vi "Measurement Logic.vi"(8 "error in":errorcluster, 9 "measurement configuration":T4={"config"="SI1", "BITFILE"=""}, 10 "measure call context in":refnum<class "Measure Call Context.lvclass">, 11 "user event out":refnum<user-event>) -> (0 "Error Out":errorcluster, 2 "measure call context out":refnum<class "Measure Call Context.lvclass">, 3 "measurement results":T1 {"BYTES ACQUIRED" format="%#.6p"})   [LabVIEW 2025, in "Automotive Vision.lvclass"]
doc: "Contains the core logic for executing the measurement."
uses:
  Automotive Vision.lvclass
  <vilib>/Plug-In SDKs/Measurements/Measure Call Context/Measure Call Context.lvclass
  <vilib>/rvi/interface/nirviCloseFPGA/nirviCloseFPGA.xnode
  Automotive Vision.lvclass/Automotive Vision.ctl
  Measurement Results.ctl
  ttashjia/GSE/Host/Acq/GettingStarted_Acq_148X_Host.lvlib
  ttashjia/GSE/Host/Common/GettingStarted_Common_148X_Host.lvlib
  <instrlib>/FlexRIO/API/Host/v1/NI FlexRIO API v1.lvlib
  <vilib>/vision/Image Controls.llb/IMAQ Image.ctl
  <instrlib>/FlexRIO/CSI-2/v2/Common/Types/LLP Data Type.ctl
  <instrlib>/FlexRIO/CSI-2/v2/Common/NI CSI-2 API Common v2.lvlib
  <vilib>/FPGAPlugInAG/Dynamic/niLvFpga_Close_Dynamic.vi
  <instrlib>/FlexRIO/API/Host/v1/NI FlexRIO/API/Wait for PoC Safe to Disconnect Channels Array.vi
  Automotive-Vision OOB Data Transfer/Automotive-Vision OOB Data Transfer.lvlib
  Measurement Configuration.ctl
panel:
  in  "Serial Channel (2nd Display)":fxp<+,3,3>
  in  "Serial Channel (1st Display)":fxp<+,3,3>
  in  "Acquired Serial Input Channel Data":T2(tab)
  out "Source Rate (fps)(1st Display)":dbl
  out "Update Rate (fps)(1st Display)":dbl
  out "1st channel display":T3(plugin-control)
  out "Bytes Acquired (1st Channel)":i64 format="%#.6p"
  out "Packets Logged (1st Channel)":i64
  out "Source Rate (fps)(2nd Display)":dbl
  out "Update Rate (fps)(2nd Display)":dbl
  out "2nd channel display":T3(plugin-control)
  out "Packets Logged (2nd Channel)":i64
  out "Bytes Acquired (2nd Channel)":i64 format="%#.6p"
  out "Acquisition In Progress":bool
  out "Acquisition Duration (s)":dbl format="%.1f"
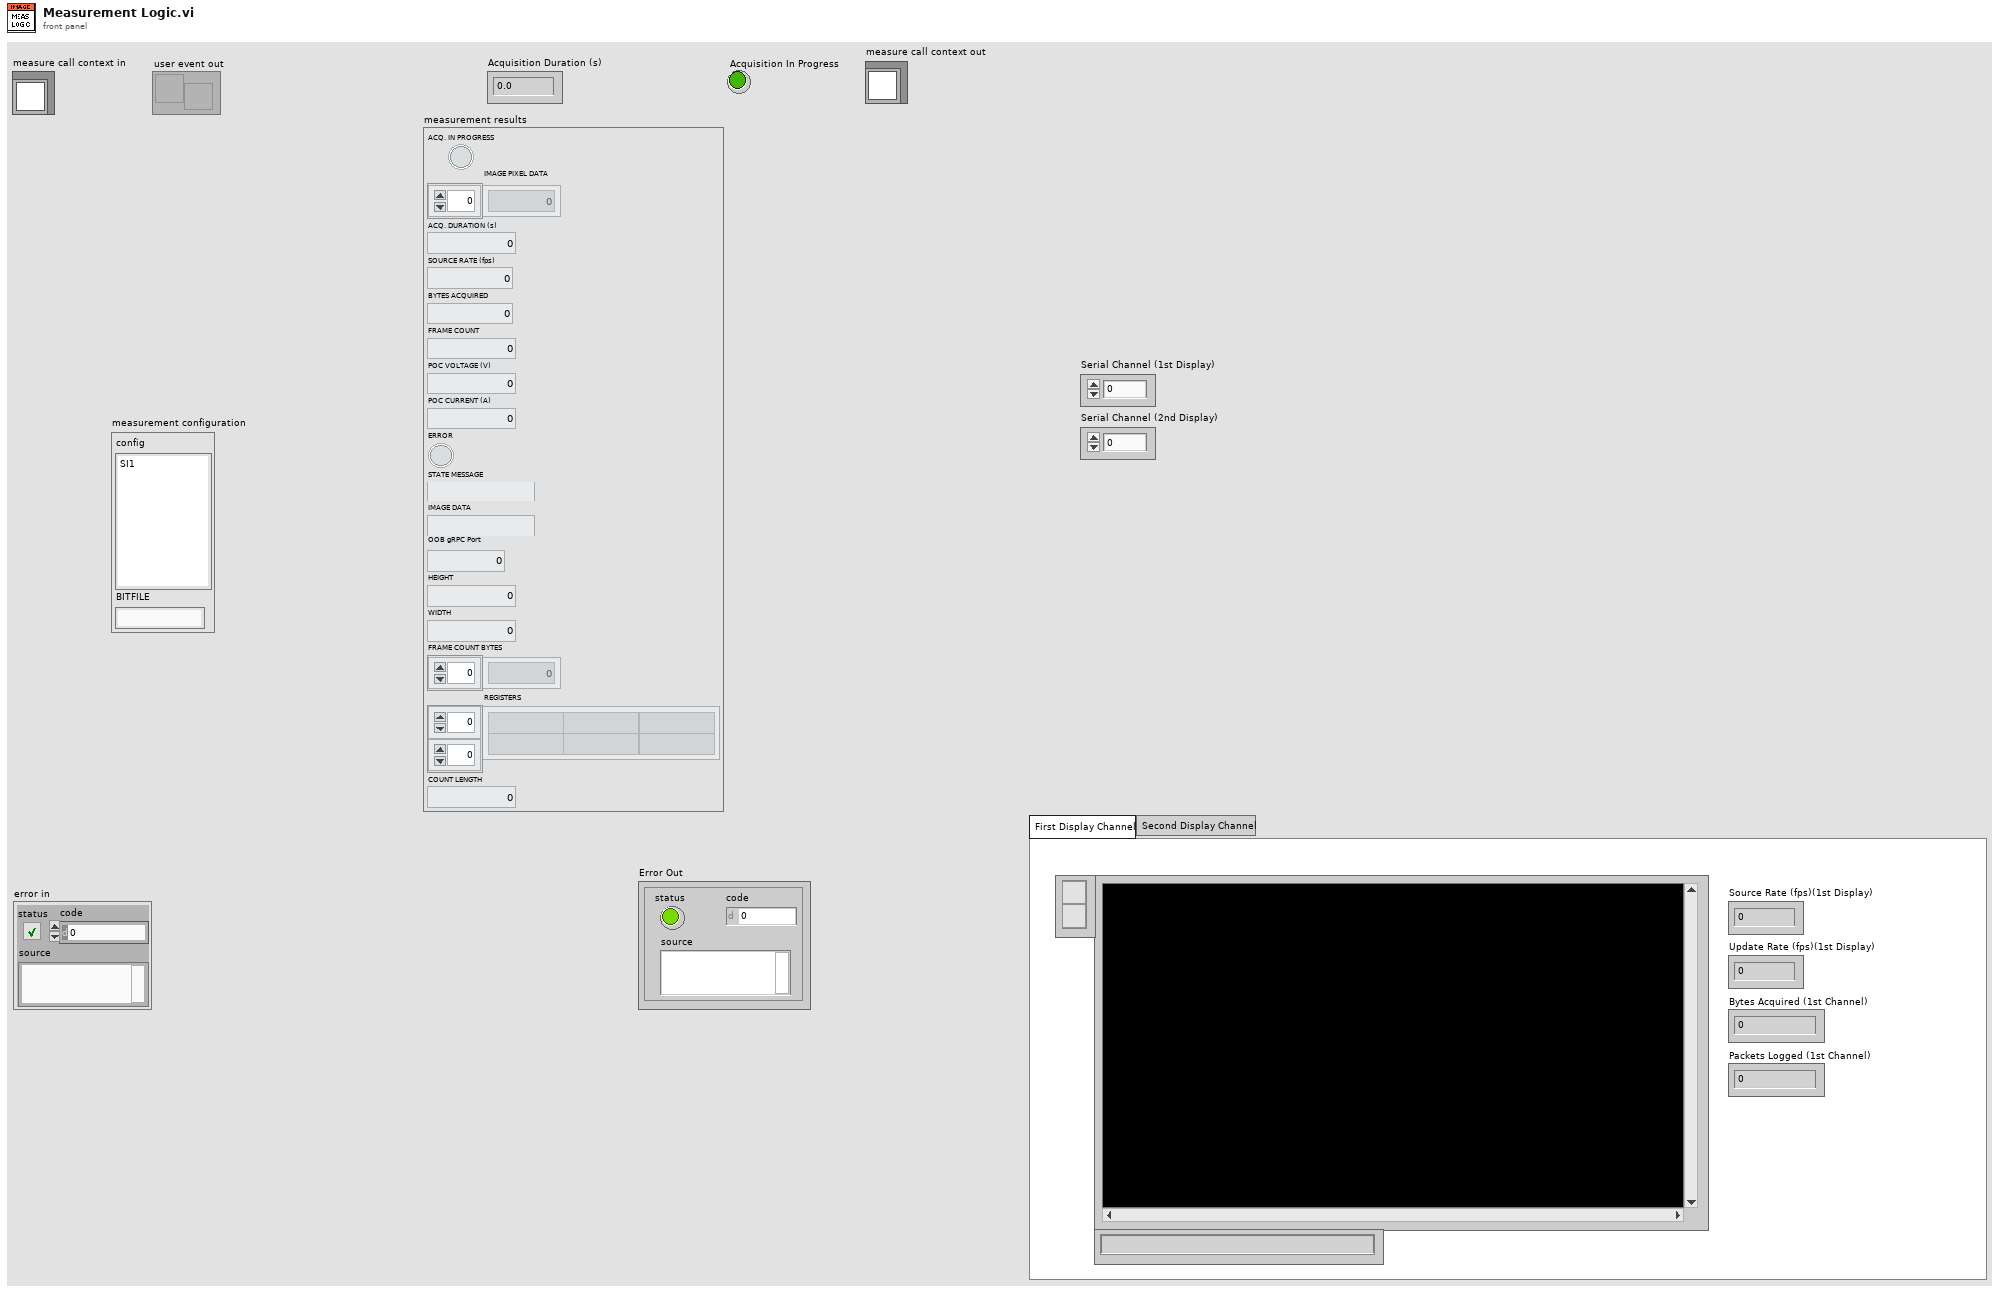
[diagram p1: front panel]
types:
  T1 = typedef "Automotive Vision.lvclass/Measurement Results.ctl" = cluster{"ACQ. IN PROGRESS":bool, "IMAGE PIXEL DATA":u32[], "ACQ. DURATION (s)":dbl, "SOURCE RATE (fps)":dbl, "BYTES ACQUIRED":u64, "FRAME COUNT":u64, "POC VOLTAGE (V)":dbl, "POC CURRENT (A)":dbl, "ERROR":bool, "STATE MESSAGE":string, "IMAGE DATA":string, "OOB gRPC Port":i32, "HEIGHT":u64, "WIDTH":u64, "FRAME COUNT BYTES":u32[], "REGISTERS":string[][], "COUNT LENGTH":u64}
  T2 = enum32{"First Display Channel", "Second Display Channel"}
  T3 = typedef "IMAQ Image.ctl" = refnum<image>
  T4 = typedef "Automotive Vision.lvclass/Measurement Configuration.ctl" = cluster{"config":string, "BITFILE":string}
  T5 = typedef "NI CSI-2 API Common v2.lvlib/LLP Data Type.ctl" = enum8{"Frame Start", "Frame End", "Line Start", "Line End", "End of Transmission", "Reserved 0", "Reserved 1", "Reserved 2", "Generic Short Packet 1", "Generic Short Packet 2", "Generic Short Packet 3", "Generic Short Packet 4", "Generic Short Packet 5", "Generic Short Packet 6", "Generic Short Packet 7", "Generic Short Packet 8", "Null", "Blanking Data", "Embedded 8-bit non Image Data", "Generic Long Packet 1", "Generic Long Packet 2", "Generic Long Packet 3", "Generic Long Packet 4", "Reserved 3", "YUV420 8-bit", "YUV420 10-bit", "Legacy YUV420 8-bit", "Reserved 4", "YUV420 8-bit Chroma Shifted", "YUV420 10-bit Chroma Shifted", "YUV422 8-bit", "YUV422 10-bit", "RGB444", "RGB555", "RGB565", "RGB666", "RGB888", "Reserved 5", "Reserved 6", "RAW 24", "RAW 6", "RAW 7", "RAW 8", "RAW 10", "RAW 12", "RAW 14", "RAW 16", "RAW 20", "User Defined 8-bit Data 1", "User Defined 8-bit Data 2", "User Defined 8-bit Data 3", "User Defined 8-bit Data 4", "User Defined 8-bit Data 5", "User Defined 8-bit Data 6", "User Defined 8-bit Data 7", "User Defined 8-bit Data 8", "USL Command", "Reserved 7", "Reserved 8", "Reserved 9", "Reserved 10", "Reserved 11", "Reserved 12", "LRTE EPD Spacer"}
  T6 = typedef "GettingStarted_Common_148X_Host.lvlib/Serial Channel Configuration.ctl" = cluster{"Serial Channel":string, "FPGA Display Parameters":T7, "RAW Display Parameters":cluster{"Interpretation":T8, "Bayer Parameters":cluster{"Pattern":i32, "Algorithm":i32, "Red Gain":dbl, "Green Gain":dbl, "Blue Gain":dbl}}}
  T7 = typedef "NI CSI-2 API FPGA v2.lvlib/Display Parameters.ctl" = cluster{"virtual channel":fxp<+,4,4>, "payload data type":T5, "frame skip count":u16, "line skip count":u8, "pixel skip count":fxp<+,5,5>}
  T8 = typedef "GettingStarted_Common_148X_Host.lvlib/RAW Interpretation for Display.ctl" = enum16{"Grayscale", "Bayer", "RGB", "YUV422", "YUV420", "Legacy YUV420"}
  T9 = typedef "Automotive Vision.lvclass/autovision_config.ctl" = cluster{"RIO Device":string, "Serial Channel":string, "SERDES Script":string, "POC Source":u32, "CSI-2 Data Source":u32, "Lane Count":u32, "Reference Clock":dbl, "Image Data Type":u32, "Interpretation":u32, "Pattern":u32, "Algorithm":u32, "Virtual Channel":u32, "Embedded Data":T10, "Registers":T12[], "Log Path":string}
  T10 = typedef "Automotive Vision.lvclass/embedded data.ctl" = cluster{"Pre-embedded Lines":dbl, "Pre-embedded Line Length":dbl, "Post-embedded Lines":dbl, "Post-embedded Line Length":dbl, "Frame Count":T11}
  T11 = typedef "Automotive Vision.lvclass/embedded data item.ctl" = cluster{"Line":dbl, "Offset":dbl, "Byte Count":dbl}
  T12 = typedef "Automotive Vision.lvclass/register.ctl" = cluster{"Name":string, "Device":u8, "Address":u16, "Min":u16, "Max":u16}
  T13 = typedef "GettingStarted_Common_148X_Host.lvlib/Serial Channel Display Parameters.ctl" = cluster{"images":cluster{"grayscale":T3, "color":T3}, "RAW parameters":cluster{"interpretation":T8, "bayer parameters":cluster{"pattern":i32, "algorithm":i32, "red gain":dbl, "green gain":dbl, "blue gain":dbl}}}
  T14 = typedef "Automotive-Vision OOB Data Transfer.lvlib/OOB to Logic Data.ctl" = cluster{"PauseResume":bool, "ExportPath":string, "ExportType":u16, "Export":bool}
  T15 = cluster{"Acquisition In Progress":refnum<vi>, "Acquisition Duration (s)":refnum<vi>, "Bytes Acquired (1st Channel)":refnum<vi>}
  T16 = typedef "Event Messenger-bool.lvlib/))Channel.ctl" = refnum<queue>
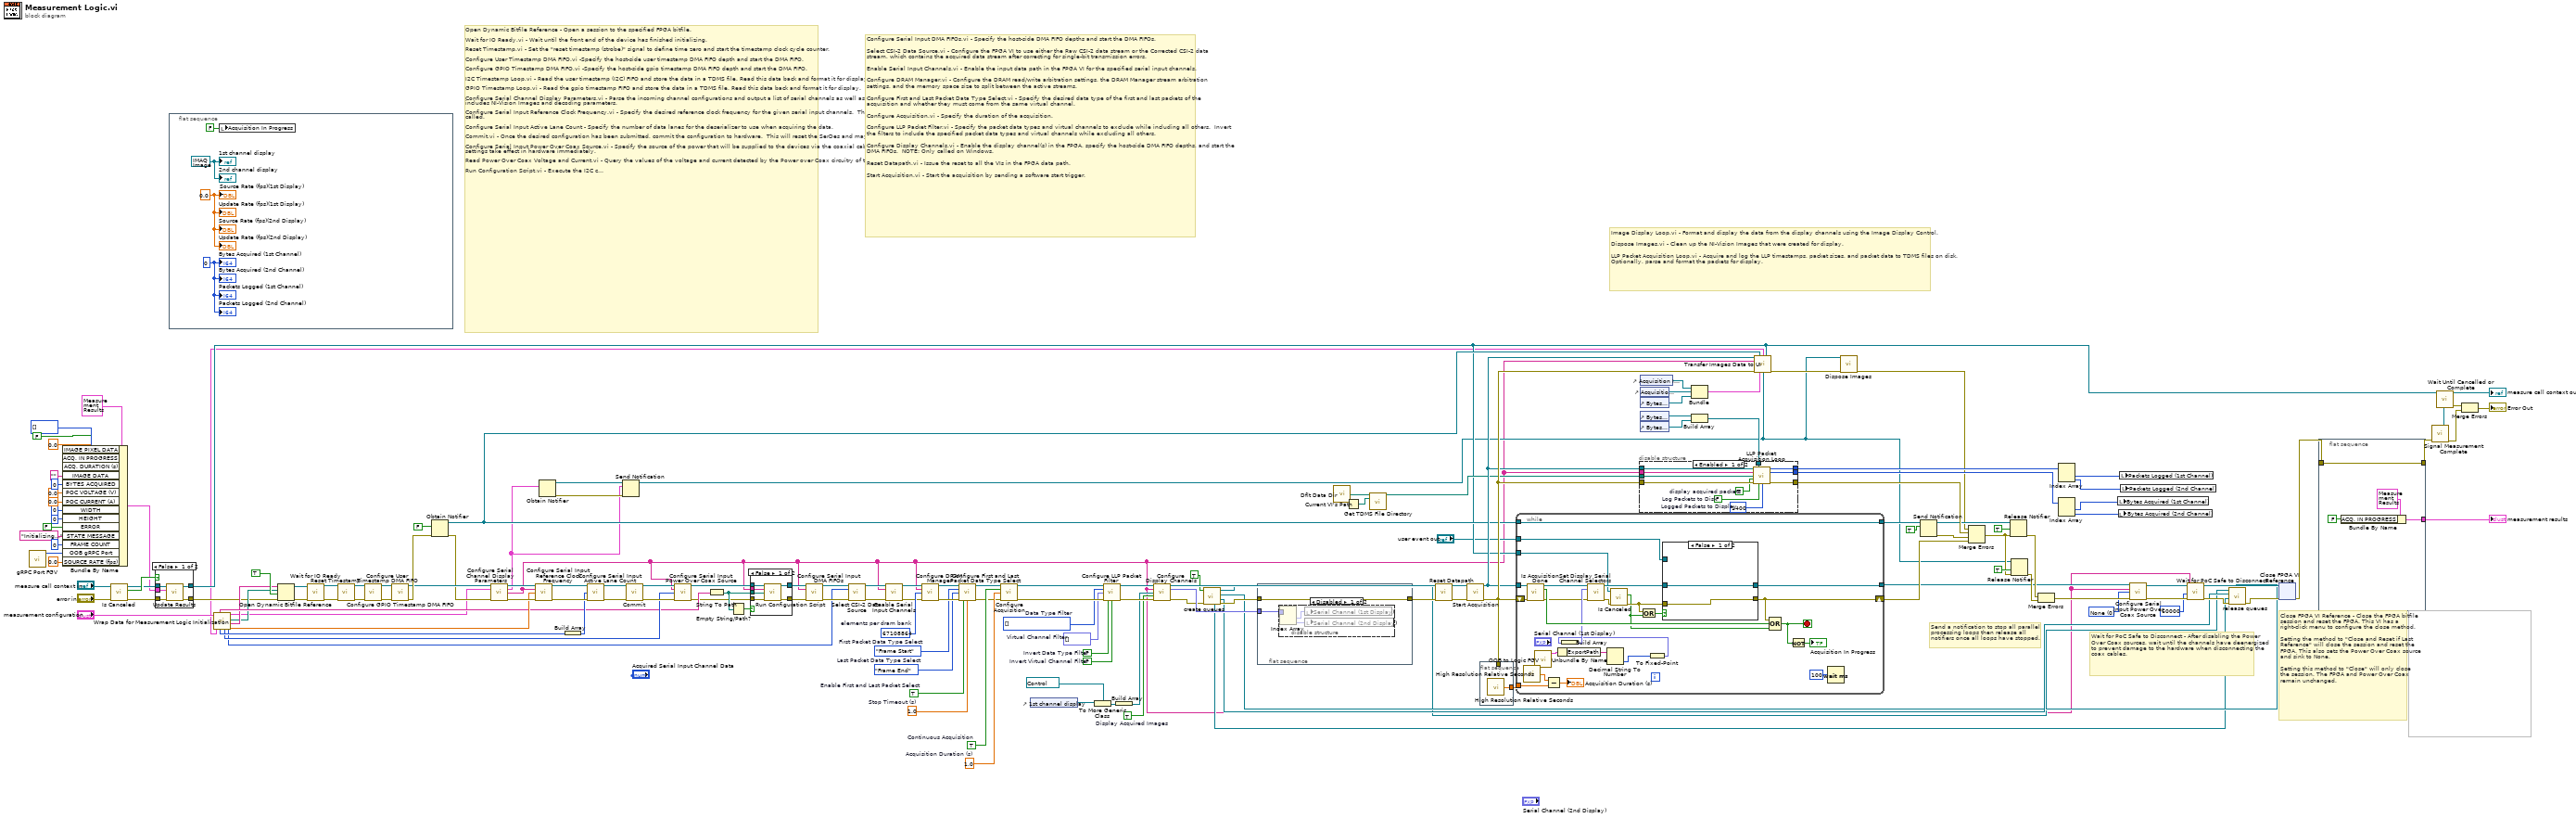
[diagram p0: block diagram]
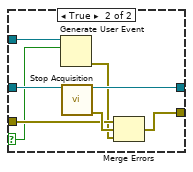
[diagram p5: hidden frame]
diagram:
  w138 = FALSE  # Invert Virtual Channel Filter
  w139 = FALSE  # Invert Data Type Filter
  w140 = fxp<+,4,4>[] []  # Virtual Channel Filter
  w106 = TRUE  # Display Acquired Images
  w143 = T5[] [] items=["Frame Start", "Frame End", "Line Start", "Line End", "End of Transmission", "Reserved 0", "Reserved 1", "Reserved 2", "Generic Short Packet 1", "Generic Short Packet 2", "Generic Short Packet 3", "Generic Short Packet 4", "Generic Short Packet 5", "Generic Short Packet 6", "Generic Short Packet 7", "Generic Short Packet 8", "Null", "Blanking Data", "Embedded 8-bit non Image Data", "Generic Long Packet 1", "Generic Long Packet 2", "Generic Long Packet 3", "Generic Long Packet 4", "Reserved 3", "YUV420 8-bit", "YUV420 10-bit", "Legacy YUV420 8-bit", "Reserved 4", "YUV420 8-bit Chroma Shifted", "YUV420 10-bit Chroma Shifted", "YUV422 8-bit", "YUV422 10-bit", "RGB444", "RGB555", "RGB565", "RGB666", "RGB888", "Reserved 5", "Reserved 6", "RAW 24", "RAW 6", "RAW 7", "RAW 8", "RAW 10", "RAW 12", "RAW 14", "RAW 16", "RAW 20", "User Defined 8-bit Data 1", "User Defined 8-bit Data 2", "User Defined 8-bit Data 3", "User Defined 8-bit Data 4", "User Defined 8-bit Data 5", "User Defined 8-bit Data 6", "User Defined 8-bit Data 7", "User Defined 8-bit Data 8", "USL Command", "Reserved 7", "Reserved 8", "Reserved 9", "Reserved 10", "Reserved 11", "Reserved 12", "LRTE EPD Spacer"]  # Data Type Filter
  w146 = 1.0  # Acquisition Duration (s)
  w149 = TRUE  # Continuous Acquisition
  w128 = 1.0  # Stop Timeout (s)
  w129 = TRUE  # Enable First and Last Packet Select
  w126 = LLP_Data_Type."Frame End"  # Last Packet Data Type Select
  w127 = LLP_Data_Type."Frame Start"  # First Packet Data Type Select
  w66 = 0 items=["None", "Internal", "Auxiliary"] ("power over coax source")
  w155 = u32 67108864  # elements per dram bank
  # "Wait for PoC Safe to Disconnect - After disabling the Power Over Coax sources, wait until the channels have deenergized to prevent damage to the hardware when disconnecting the coax cables."
  # "Send a notification to stop all parallel processing loops then release all notifiers once all loops have stopped."
  # "Image Display Loop.vi - Format and display the data from the display channels using the Image Display Control.   \n\nDispose Images.vi - Clean up the NI-Vision Images that were created for display.\n\nLLP Packet Acquisition Loop.vi - Acquire and log the LLP timestamps, packet sizes, and packet data to TDMS files on disk.  Optionally, parse and format the packets for display."
  # "Configure Serial Input DMA FIFOs.vi - Specify the host-side DMA FIFO depths and start the DMA FIFOs.\n\nSelect CSI-2 Data Source.vi - Configure the FPGA VI to use either the Raw CSI-2 data stream or the Corrected CSI-2 data stream, which contains the acquired data stream after correcting for single-bit transmission errors.\n\nEnable Serial Input Channels.vi - Enable the input data path in the FPGA VI for the specified serial input channels.\n\nConfigure DRAM Manager.vi - Configure the DRAM read/write arbitration settings, the DRAM Manager stream arbitration settings, and the memory space size to split between the active streams.\n\nConfigure First and Last Packet Data Type Select.vi - Specify the desired data type of the first and last packets of the acquisition and whether they must come from the same virtual channel.\n\nConfigure Acquisition.vi - Specify the duration of the acquisition.\n\nConfigure LLP Packet Filter.vi - Specify the packet data types and virtual channels to exclude while including all others.  Invert the filters to include the specified packet data types and virtual channels while excluding all others.\n\nConfigure Display Channels.vi - Enable the display channel(s) in the FPGA, specify the host-side DMA FIFO depths, and start the DMA FIFOs.  NOTE: Only called on Windows. \n\nReset Datapath.vi - Issue the reset to all the VIs in the FPGA data path.\n\nStart Acquisition.vi - Start the acquisition by sending a software start trigger."
  # "Close FPGA VI Reference - Close the FPGA bitfile session and reset the FPGA. This VI has a right-click menu to configure the close method. \n\nSetting the method to \"Close and Reset if Last Reference\" will close the session and reset the FPGA. This also sets the Power Over Coax source and sink to None.\n\nSetting this method to \"Close\" will only close the session. The FPGA and Power Over Coax remain unchanged."
  # "Open Dynamic Bitfile Reference - Open a session to the specified FPGA bitfile.\n\nWait for IO Ready.vi - Wait until the front end of the device has finished initializing.\n\nReset Timestamp.vi - Set the \"reset timestamp (strobe)\" signal to define time zero and start the timestamp clock cycle counter.\n\nConfigure User Timestamp DMA FIFO.vi -Specify the host-side user timestamp DMA FIFO depth and start the DMA FIFO.\n\nConfigure GPIO Timestamp DMA FIFO.vi -Specify the host-side gpio timestamp DMA FIFO depth and start the DMA FIFO.\n\nI2C Timestamp Loop.vi - Read the user timestamp (I2C) FIFO and store the data in a TDMS file. Read this data back and format it for display.\n\nGPIO Timestamp Loop.vi - Read the gpio timestamp FIFO and store the data in a TDMS file. Read this data back and format it for display.\n\nConfigure Serial Channel Display Parameters.vi - Parse the incoming channel configurations and output a list of serial channels as well as a list of serial channel display parameters, which includes NI-Vision Images and decoding parameters.\n\nConfigure Serial Input Reference Clock Frequency.vi - Specify the desired reference clock frequency for the given serial input channels.  These settings do not take effect until Commit.vi is called.\n\nConfigure Serial Input Active Lane Count - Specify the number of data lanes for the deserializer to use when acquiring the data. \n\nCommit.vi - Once the desired configuration has been submitted, commit the configuration to hardware.  This will reset the SerDes and may cause GPIO lines to toggle. \n\nConfigure Serial Input Power Over Coax Source.vi - Specify the source of the power that will be supplied to the devices via the coaxial cables attached to the given serial input channels.  These settings take effect in hardware immediately.\n\nRead Power Over Coax Voltage and Current.vi - Query the values of the voltage and current detected by the Power over Coax circuitry of the given serial channels.\n\nRun Configuration Script.vi - Execute the I2C commands in the specified script file for the given serial channels.  The script is used to configure the serializer, deserializer, or other I2C slave device, such as the image sensor."
  n1 = call "gRPC Port FGV.vi"() -> ("Listening Port out"=w39:i32)  [unwired: 11 in]
  n2 = Bundle By Name(cluster=T1 {"ACQ. IN PROGRESS"=FALSE, "IMAGE PIXEL DATA"=[], "ACQ. DURATION (s)"=0.0, "SOURCE RATE (fps)"=0.0, "BYTES ACQUIRED"=0, "FRAME COUNT"=0, "POC VOLTAGE (V)"=0.0, "POC CURRENT (A)"=0.0, "ERROR"=FALSE, "STATE MESSAGE"="", "IMAGE DATA"="", "OOB gRPC Port"=0, "HEIGHT"=0, "WIDTH"=0, "FRAME COUNT BYTES"=[], "REGISTERS"=[], "COUNT LENGTH"=0} ("Measurement Results"), "IMAGE PIXEL DATA"=u32[] [], "ACQ. IN PROGRESS"=FALSE, "ACQ. DURATION (s)"=0.0, "IMAGE DATA"="", "BYTES ACQUIRED"=u64 0, "POC VOLTAGE (V)"=0.0, "POC CURRENT (A)"=0.0, "WIDTH"=u64 0, "HEIGHT"=u64 0, "ERROR"=FALSE, "STATE MESSAGE"="Initializing...", "FRAME COUNT"=u64 0, "OOB gRPC Port"=w39, "SOURCE RATE (fps)"=0.0) -> (w35:T1)
  n3 = call <vilib>:"Is Canceled.vi"("error in"="error in", "measure call context in"="measure call context in") -> ("error out"=w38:errorcluster, "is canceled?"=w37:bool, "measure call context out"=w36:refnum<class "Measure Call Context.lvclass">)  [unwired: 7 in]
  n4 = case shown="False" w37 {
    tunnel: w35 -> [w164 _]
    tunnel: [w163 w166] -> w32
    tunnel: w36 -> [w162 w165]
    tunnel: w38 -> [w161 w166]
    tunnel: [w160 w165] -> w17
    frame False {
      n5 = call <vilib>:"Update Results.vi"("error in"=w161, "measurement results"=w164, "measure call context in"=w162) -> ("error out"=w163:errorcluster, "measure call context out"=w160:refnum<class "Measure Call Context.lvclass">)  [unwired: 7 in]
    }
    frame True {
    }
  }
  n6 = flat-sequence {
    frame #0 {
      w168 = i64 0 ("Number of Packets Acquired (1st Channel)")
      w169 = 0.0 ("display fps (2nd display)")
      w170 = T3 refnum ("first channel display")
      n7 = local write "Acquisition In Progress"(FALSE ("Acquisition In Progress")) -> ()
      "1st channel display" <- w170
      "2nd channel display" <- w170
      "Update Rate (fps)(1st Display)" <- w169
      "Update Rate (fps)(2nd Display)" <- w169
      "Packets Logged (1st Channel)" <- w168
      "Packets Logged (2nd Channel)" <- w168
      "Source Rate (fps)(1st Display)" <- w169
      "Source Rate (fps)(2nd Display)" <- w169
      "Bytes Acquired (1st Channel)" <- w168
      "Bytes Acquired (2nd Channel)" <- w168
    }
  }
  n8 = call "Wrap Data for Measurement Logic Initialization.vi"("measurement configuration"="measurement configuration") -> ("REF. CLOCK  (Hz)"=w56:dbl, "RIO HANDLER"=w52:string, "CSI-2 DATA SOURCE"=w57:u32, "Serial Input Configuration"=w2:T6[], "POC SOURCE"=w58:u32, "appended path"=w51:path, "SI ACTIVE LANE CNT"=w59:u32, "PATH TO CONFIGURATION SCRIPT"=w55:string, "config"=w11:T9)  [unwired: 2 in]
  n9 = Open Dynamic Bitfile Reference(0:w52, 1:w51, 2:TRUE ("Run When Loaded"), 3:w32) -> (5:w141:refnum<k20>, 8:w46:errorcluster)  [unwired: 1 in]
  n10 = call <instrlib>:"Wait for IO Ready.vi"("fpga interface in"=w141, "error in"=w46) -> ("fpga interface out"=w103:refnum<k20>, "error out"=w104:errorcluster)  [unwired: 10 in, 2 out]
  n11 = call "Reset Timestamp.vi"("fpga interface in"=w103, "error in (no error)"=w104) -> ("fpga interface out"=w93:refnum<k20>, "error out"=w92:errorcluster)  [unwired: 12 in]
  n12 = call "Configure User Timestamp DMA FIFO.vi"("fpga interface in"=w93, "error in (no error)"=w92) -> ("fpga interface out"=w91:refnum<k20>, "error out"=w90:errorcluster)  [unwired: 12 in]
  n13 = call "Configure GPIO Timestamp DMA FIFO.vi"("fpga interface in"=w91, "error in (no error)"=w90) -> ("fpga interface out"=w87:refnum<k20>, "error out"=w89:errorcluster)  [unwired: 12 in]
  n14 = Obtain Notifier(notification data type=FALSE ("result"), error in (no error)=w89) -> (notifier out=w77:refnum<notifier>, error out=w86:errorcluster)  [unwired: 2 in, 1 out]
  n15 = call "Configure Serial Channel Display Parameters.vi"("fpga interface in"=w87, "serial channel configurations"=w2, "error in (no error)"=w86) -> ("fpga interface out"=w118:refnum<k20>, "serial channel display parameters"=w74:T13[], "serial channels"=w1:string[], "error out"=w117:errorcluster)  [unwired: 9 in]
  n16 = call "Configure Serial Input Reference Clock Frequency.vi"("fpga interface in"=w118, "serial input channels"=w1, "serial input reference clock frequency (Hz)"=w56, "error in (no error)"=w117) -> ("fpga interface out"=w82:refnum<k20>, "error out"=w81:errorcluster)  [unwired: 10 in]
  n17 = Obtain Notifier(notification data type=w74) -> (notifier out=w76:refnum<notifier>, error out=w75:errorcluster)  [unwired: 3 in, 1 out]
  n18 = Build Array(w59) -> (w78:u32[])
  n19 = call "Configure Serial Input Active Lane Count.vi"("fpga interface in"=w82, "serial input active lane counts"=w78, "error in (no error)"=w81) -> ("fpga interface out"=w80:refnum<k20>, "error out"=w79:errorcluster)  [unwired: 11 in]
  n20 = Send Notification(notification=w74, notifier=w76, error in (no error)=w75) -> (notifier out=w16:refnum<notifier>)  [unwired: 1 out]
  n21 = call <instrlib>:"Commit.vi"("fpga interface in"=w80, "error in"=w79) -> ("fpga interface out"=w144:refnum<k20>, "error out"=w145:errorcluster)  [unwired: 12 in]
  n22 = call "Configure Serial Input Power Over Coax Source.vi"("fpga interface in"=w144, "serial input channels"=w1, "power over coax source"=w58, "error in (no error)"=w145) -> ("fpga interface out"=w41:refnum<k20>, "error out"=w40:errorcluster)  [unwired: 9 in, 1 out]
  n23 = String To Path(string=w55) -> (path=w54:path)
  n24 = Empty String/Path?(string/path=w54) -> (empty?=w105:bool)
  n25 = case shown="False" w105 {
    tunnel: [w176 w177] -> w153
    tunnel: [w175 w178] -> w148
    tunnel: w40 -> [w174 w177]
    tunnel: w41 -> [w173 w178]
    tunnel: w1 -> [w172 _]
    tunnel: w54 -> [w171 _]
    frame False {
      n26 = call "Run Configuration Script.vi"("fpga interface in"=w173, "serial channels"=w172, "configuration script"=w171, "error in (no error)"=w174) -> ("fpga interface out"=w175:refnum<k20>, "error out"=w176:errorcluster)  [unwired: 10 in]
    }
    frame True {
    }
  }
  n27 = call "Configure Serial Input DMA FIFOs.vi"("fpga interface in"=w148, "serial channels"=w1, "error in (no error)"=w153) -> ("fpga interface out"=w137:refnum<k20>, "error out"=w134:errorcluster)  [unwired: 11 in]
  n28 = call "Select CSI-2 Data Source.vi"("fpga interface in"=w137, "csi-2 data source"=w57, "error in (no error)"=w134) -> ("fpga interface out"=w136:refnum<k20>, "error out"=w135:errorcluster)  [unwired: 11 in]
  n29 = call "Enable Serial Input Channels.vi"("fpga interface in"=w136, "serial input channels"=w1, "error in (no error)"=w135) -> ("fpga interface out"=w147:refnum<k20>, "error out"=w154:errorcluster)  [unwired: 11 in]
  n30 = call "Configure DRAM Manager.vi"("fpga interface in"=w147, "serial channels"=w1, "elements per dram bank"=w155, "error in (no error)"=w154) -> ("fpga interface out"=w130:refnum<k20>, "error out"=w133:errorcluster)  [unwired: 10 in]
  n31 = call "Configure First and Last Packet Data Type Select.vi"("fpga interface in"=w130, "first packet data type select"=w127, "last packet data type select"=w126, "error in (no error)"=w133, "enable first and last packet select"=w129, "stop timeout (s)"=w128) -> ("fpga interface out"=w131:refnum<k20>, "error out"=w132:errorcluster)  [unwired: 8 in]
  n32 = call "Configure Acquisition.vi"("fpga interface in"=w131, "continuous acquisition (T)"=w149, "acquisition duration (s)"=w146, "error in (no error)"=w132) -> ("fpga interface out"=w150:refnum<k20>, "error out"=w151:errorcluster)  [unwired: 10 in]
  n33 = control-ref of="1st channel display"() -> (w43:refnum<vi>)
  n34 = To More Generic Class(target class=refnum<vi> refnum ("image display reference"), reference=w43) -> (generic class reference=w45:refnum<vi>)
  n35 = call "Configure LLP Packet Filter.vi"("fpga interface in"=w150, "data type filter"=w143, "virtual channel filter"=w140, "error in (no error)"=w151, "invert data type filter"=w139, "invert virtual channel filter"=w138) -> ("fpga interface out"=w119:refnum<k20>, "error out"=w116:errorcluster)  [unwired: 8 in]
  n36 = Build Array(w45) -> (w42:refnum<vi>[])
  n37 = call "Configure Display Channels.vi"("fpga interface in"=w119, "serial channels"=w1, "display references in"=w42, "enable image display"=w106, "error in (no error)"=w116) -> ("fpga interface out"=w115:refnum<k20>, "display serial channels"=w114:fxp<+,3,3>[], "error out"=w12:errorcluster)  [unwired: 7 in, 1 out]
  n38 = call "create queues.vi"("error in (no error)"=w12, "create if not found? (T)"=TRUE) -> ("error out"=w10:errorcluster, "i2c queue out"=w6:refnum<queue>, "power monitor queue out"=w5:refnum<queue>, "image queue out"=w4:refnum<queue>, "register monitor queue out"=w3:refnum<queue>)  [unwired: 5 in]
  n39 = flat-sequence {
    tunnel: w114 -> [w180]
    tunnel: w10 -> [w179]
    tunnel: [w179] -> w113
    frame #0 {
      n40 = disable-structure shown="Disabled" {
        disable-tunnel: w180 -> [w183 _]
        frame Disabled {
          n41 = Index Array(array=w183) -> (element #1=w182:fxp<+,3,3>, element #2=w181:fxp<+,3,3>)  [unwired: 2 in]
          n42 = local write "Serial Channel (1st Display)"(w182) -> ()
          n43 = local write "Serial Channel (2nd Display)"(w181) -> ()
        }
        frame Enabled {
        }
      }
    }
  }
  n44 = call <vilib>:"Dflt Data Dir.vi"() -> ("App:Default Data Directory"=w53:path)
  n45 = Current VI's Path() -> (path=w122:path)
  n46 = call "Get TDMS File Directory.vi"("tdms file directory in"=w53, "calling vi path"=w122) -> ("tdms file directory out"=w85:path)  [unwired: 13 in]
  n47 = call "Reset Datapath.vi"("fpga interface in"=w115, "error in (no error)"=w113) -> ("fpga interface out"=w152:refnum<k20>, "error out"=w88:errorcluster)  [unwired: 12 in]
  n48 = call "Start Acquisition.vi"("fpga interface in"=w152, "error in (no error)"=w88) -> ("fpga interface out"=w101:refnum<k20>, "error out"=w102:errorcluster)  [unwired: 12 in]
  n49 = flat-sequence {
    tunnel: [w184] -> w123
    tunnel: w102 -> [_]
    frame #0 {
      n50 = call <vilib>:"High Resolution Relative Seconds.vi"() -> ("relative seconds"=w184:dbl)
    }
  }
  n51 = while {
    shift-right: [w192] -> w83
    shift-left: w102 -> [w203]
    tunnel: w101 -> [w205]
    tunnel: w123 -> [w207]
    tunnel: w77 -> [w202]
    tunnel: [w202] -> w98
    tunnel: [w193] -> w69
    tunnel: w17 -> [w199]
    tunnel: "user event out" -> [w189]
    stop <- w204 stop-if-true
    n52 = call <vilib>:"High Resolution Relative Seconds.vi"() -> ("relative seconds"=w208:dbl)
    n53 = call "Is Acquisition Done.vi"("fpga interface in"=w205, "error in (no error)"=w203) -> ("fpga interface out"=w195:refnum<k20>, "acquisition done"=w210:bool, "error out"=w194:errorcluster)  [unwired: 11 in]
    n54 = call "OOB to Logic FGV.vi"() -> ("OOB to Logic Data out"=w188:T14)  [unwired: 10 in, 1 out]
    n55 = Subtract(x=w208, y=w207) -> (x-y=→"Acquisition Duration (s)":dbl)
    n56 = Unbundle By Name(w188) -> ("ExportPath"=w187:string)
    n57 = Decimal String To Number(string=w187) -> (number=w186:i32)  [unwired: 2 in, 1 out]
    n58 = To Fixed-Point(number=w186) -> (fixed-point=w185:fxp<+/-,32,32>)  [unwired: 1 in]
    n59 = Build Array(w185) -> (w206:fxp<+/-,32,32>[])
    n60 = call "Set Display Serial Channel Selectors.vi"("fpga interface in"=w195, "display serial channel selectors"=w206, "error in (no error)"=w194) -> ("fpga interface out"=w200:refnum<k20>, "error out"=w201:errorcluster)  [unwired: 11 in]
    n61 = call <vilib>:"Is Canceled.vi"("error in"=w201, "measure call context in"=w199) -> ("error out"=w197:errorcluster, "is canceled?"=w191:bool)  [unwired: 7 in, 1 out]
    n62 = Compound Arithmetic op=OR(w197, w191) -> (w190:bool)
    n63 = case shown="False" w190 {
      selector: w190 -> [_ w214]
      tunnel: [w212 w217] -> w192
      tunnel: w197 -> [w212 w216]
      tunnel: [w211 w219] -> w193
      tunnel: w200 -> [w211 w218]
      tunnel: w189 -> [_ w215]
      frame False {
      }
      frame True {
        n64 = Generate User Event(user event=w215, event data cluster=w214) -> (error out=w213:errorcluster)  [unwired: 2 in, 1 out]
        n65 = call "Stop Acquisition.vi"("fpga interface in"=w218) -> ("fpga interface out"=w219:refnum<k20>, "error out"=w220:errorcluster)  [unwired: 13 in]
        n66 = Merge Errors(w216, w220, w213) -> (w217:errorcluster)
      }
    }
    n67 = Compound Arithmetic op=OR(w192, w210, w191) -> (w204:bool)
    n68 = Not(x=w204) -> (.not. x?=→"Acquisition In Progress":bool)
    n69 = Wait (ms)(milliseconds to wait=u32 100) -> ()  [unwired: 1 out]
  }
  n70 = control-ref of="Acquisition In Progress"() -> (w50:refnum<vi>)
  n71 = control-ref of="Acquisition Duration (s)"() -> (w49:refnum<vi>)
  n72 = control-ref of="Bytes Acquired (1st Channel)"() -> (w48:refnum<vi>)
  n73 = control-ref of="Bytes Acquired (1st Channel)"() -> (w125:refnum<vi>)
  n74 = control-ref of="Bytes Acquired (2nd Channel)"() -> (w124:refnum<vi>)
  n75 = Bundle("Acquisition In Progress"=w50, "Acquisition Duration (s)"=w49, "Bytes Acquired (1st Channel)"=w48) -> (w47:T15)  [unwired: 1 in]
  n76 = Build Array(w125, w124) -> (w121:refnum<vi>[])
  n77 = disable-structure shown="Enabled" {
    disable-tunnel: w121 -> [w231 _]
    disable-tunnel: [w230 _] -> w120
    disable-tunnel: [w228 _] -> w109
    disable-tunnel: w102 -> [w227 w232]
    disable-tunnel: w101 -> [w226 _]
    disable-tunnel: [w225 w232] -> w99
    disable-tunnel: w85 -> [w224 _]
    disable-tunnel: w1 -> [w221 _]
    frame Enabled {
      w222 = i64 1400  # Logged Packets to Display
      w229 = FALSE  # Log Packets to Disk
      w223 = TRUE  # display acquired packets
      n78 = call "LLP Packet Acquisition Loop.vi"("fpga interface in"=w226, "bytes acquired references"=w231, "Serial Channels"=w221, "tdms file directory"=w224, "display acquired packets"=w223, "error in"=w227, "log to disk"=w229, "num packets to read"=w222) -> ("number of packets acquired"=w230:i64[], "number of bytes acquired"=w228:i64[], "error out"=w225:errorcluster)  [unwired: 4 in, 1 out]
    }
    frame Disabled {
    }
  }
  n79 = call "Transfer Images Data to UI.vi"("fpga interface in"=w101, "'stop' notifier"=w77, "Auto Vision Config"=w11, "measure call context in"=w17, "Active Channel"=w1, "error in"=w102, "References"=w47, "raw display notifier"=w16) -> ("error out"=w110:errorcluster)  [unwired: 6 in, 1 out]
  n80 = call "Dispose Images.vi"("raw display notifier"=w16, "error in (no error)"=w110) -> ("error out"=w84:errorcluster)  [unwired: 13 in]
  n81 = Send Notification(notification=TRUE, notifier=w98) -> (notifier out=w97:refnum<notifier>, error out=w96:errorcluster)  [unwired: 1 in]
  n82 = Merge Errors(w84, w99, w96, w83) -> (w72:errorcluster)
  n83 = Release Notifier(notifier=w97, force destroy? (F)=TRUE, error in (no error)=w72) -> (error out=w71:errorcluster)  [unwired: 2 out]
  n84 = Release Notifier(notifier=w16, force destroy? (F)=TRUE, error in (no error)=w72) -> (error out=w70:errorcluster)  [unwired: 2 out]
  n85 = Merge Errors(w71, w70) -> (w68:errorcluster)
  n86 = Index Array(array=w120) -> (element #1=w112:i64, element #2=w111:i64)  [unwired: 2 in]
  n87 = Index Array(array=w109) -> (element #1=w108:i64, element #2=w107:i64)  [unwired: 2 in]
  n88 = local write "Bytes Acquired (1st Channel)"(w108) -> ()
  n89 = local write "Bytes Acquired (2nd Channel)"(w107) -> ()
  n90 = local write "Packets Logged (1st Channel)"(w112) -> ()
  n91 = local write "Packets Logged (2nd Channel)"(w111) -> ()
  n92 = call "Configure Serial Input Power Over Coax Source.vi"("fpga interface in"=w69, "serial input channels"=w1, "power over coax source"=w66, "error in (no error)"=w68) -> ("fpga interface out"=w64:refnum<k20>, "error out"=w65:errorcluster)  [unwired: 9 in, 1 out]
  n93 = call-poly <instrlib>:"Wait for PoC Safe to Disconnect.vi"("error in"=w65, "Timeout (ms)"=60000 ("Wait for Safe to Disconnect Timeout (ms)"), "Channels"=w1, "fpga interface in"=w64) -> ("error out"=w8:errorcluster, "fpga interface out"=w67:refnum<k20>)  [unwired: 6 in]
  n94 = call "release queues.vi"("power monitor queue out"=w5, "error in (no error)"=w8, "register monitor queue out"=w3, "i2c queue out"=w6, "image queue out"=w4) -> ("error out"=w7:errorcluster)  [unwired: 6 in]
  n95 = xnode ("Close FPGA VI Reference")("FPGA VI Reference In"=w67, "error in"=w7) -> ("error out"=w60:errorcluster)
  n96 = flat-sequence {
    tunnel: [w235] -> w61
    tunnel: w60 -> [w233]
    tunnel: [w233] -> w15
    frame #0 {
      n97 = Bundle By Name(cluster=T1 {"ACQ. IN PROGRESS"=FALSE, "IMAGE PIXEL DATA"=[], "ACQ. DURATION (s)"=0.0, "SOURCE RATE (fps)"=0.0, "BYTES ACQUIRED"=0, "FRAME COUNT"=0, "POC VOLTAGE (V)"=0.0, "POC CURRENT (A)"=0.0, "ERROR"=FALSE, "STATE MESSAGE"="", "IMAGE DATA"="", "OOB gRPC Port"=0, "HEIGHT"=0, "WIDTH"=0, "FRAME COUNT BYTES"=[], "REGISTERS"=[], "COUNT LENGTH"=0} ("Measurement Results"), "ACQ. IN PROGRESS"=FALSE) -> (w235:T1)
    }
  }
  n98 = call "Signal Measurement Complete.vi"("error in (no error)"=w15) -> ("error out"=w157:errorcluster, "done channel"=w158:T16)  [unwired: 9 in]
  n99 = call "Wait Until Cancelled or Complete.vi"("done channel"=w158, "measure call context in"=w17) -> ("error out"=w156:errorcluster, "measure call context out"=→"measure call context out":refnum<class "Measure Call Context.lvclass">)  [unwired: 8 in]
  n100 = Merge Errors(w156, w157) -> (→"Error Out":errorcluster)
  "measurement results" <- w61
